vi "Simulate Market Tick.vi"(11 "market":T1) -> (3 "market out":T1)   [LabVIEW 2020, in "Full Featured MCP Server.lvlib"]
doc: "Simulates one second of the market: the mood drifts, news may break, stories start and move on, a company may report its numbers, and then all prices move. This is the whole engine in one line; each step is a VI of its own."
uses:
  Full Featured MCP Server.lvlib
  Market State.ctl
  News Item.ctl
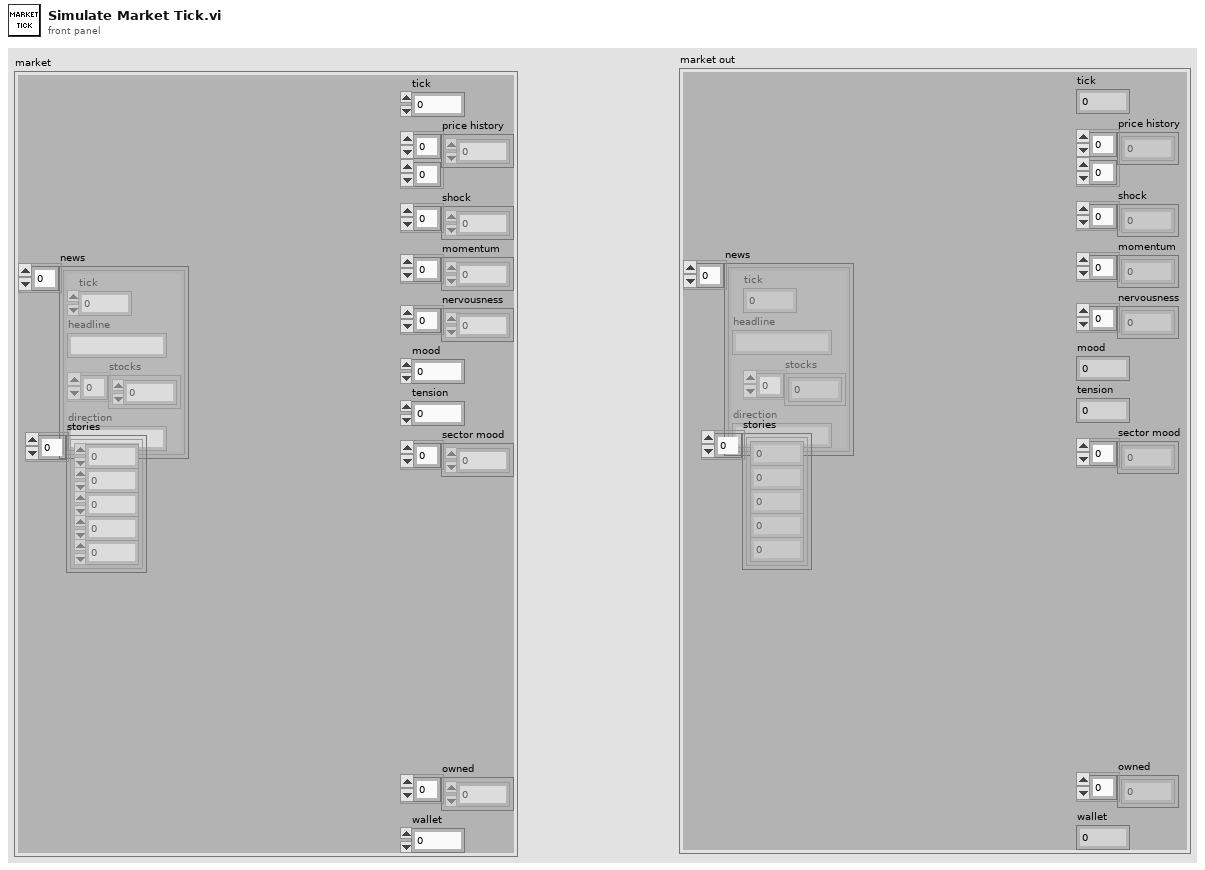
[diagram p1: front panel]
types:
  T1 = typedef "Full Featured MCP Server.lvlib/Market State.ctl" = cluster{"tick":i32, "price history":dbl[][], "shock":dbl[], "momentum":dbl[], "nervousness":dbl[], "mood":dbl, "tension":dbl, "sector mood":dbl[], "news":T2[], "stories":cluster{"arc":i32, "step":i32, "due":i32, "stock":i32, "other":i32}[], "owned":i32[], "wallet":dbl}
  T2 = typedef "Full Featured MCP Server.lvlib/News Item.ctl" = cluster{"tick":i32, "headline":string, "stocks":i32[], "direction":string}
  T3 = cluster{"tick":i32, "price history":dbl[][], "shock":dbl[], "momentum":dbl[], "nervousness":dbl[], "mood":dbl, "tension":dbl, "sector mood":dbl[], "news":cluster{"tick":i32, "headline":string, "stocks":i32[], "direction":string}[], "stories":cluster{"arc":i32, "step":i32, "due":i32, "stock":i32, "other":i32}[], "owned":i32[], "wallet":dbl}
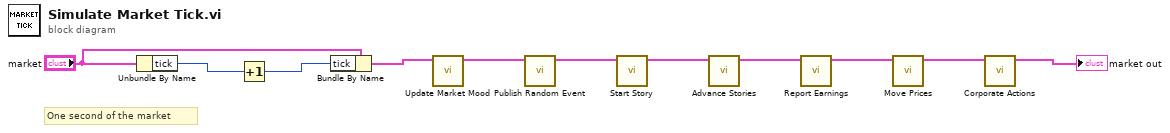
[diagram p0: block diagram]
diagram:
  # "One second of the market"
  n1 = Unbundle By Name("market") -> ("tick"=w2:i32)
  n2 = Increment(x=w2) -> (x+1=w3:i32)
  n3 = Bundle By Name(cluster="market", "tick"=w3) -> (w4:T1)
  n4 = call "Update Market Mood.vi"("market"=w4) -> ("market out"=w5:T3)  [unwired: 10 in]
  n5 = call "Publish Random Event.vi"("market"=w5) -> ("market out"=w6:T1)  [unwired: 10 in]
  n6 = call "Start Story.vi"("market"=w6) -> ("market out"=w7:T3)  [unwired: 10 in]
  n7 = call "Advance Stories.vi"("market"=w7) -> ("market out"=w8:T1)  [unwired: 10 in]
  n8 = call "Report Earnings.vi"("market"=w8) -> ("market out"=w9:T1)  [unwired: 10 in]
  n9 = call "Move Prices.vi"("market"=w9) -> ("market out"=w10:T1)  [unwired: 10 in]
  n10 = call "Corporate Actions.vi"("market"=w10) -> ("market out"=→"market out":T1)  [unwired: 10 in]
